vi "recurse property bag for specific properties.vi"(7 "hierarchy path":string, 10 "search key (match pattern)":string, 11 "property bag":refnum<k7>) -> (2 "matching properties":refnum<k7>[](array[refnum]), 3 "Report Text":string)   [LabVIEW 2020, in "nominal teststand model sequence support.lvlib"]
uses:
  nominal teststand model sequence support.lvlib
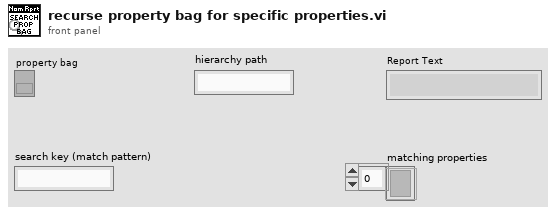
[diagram p1: front panel]
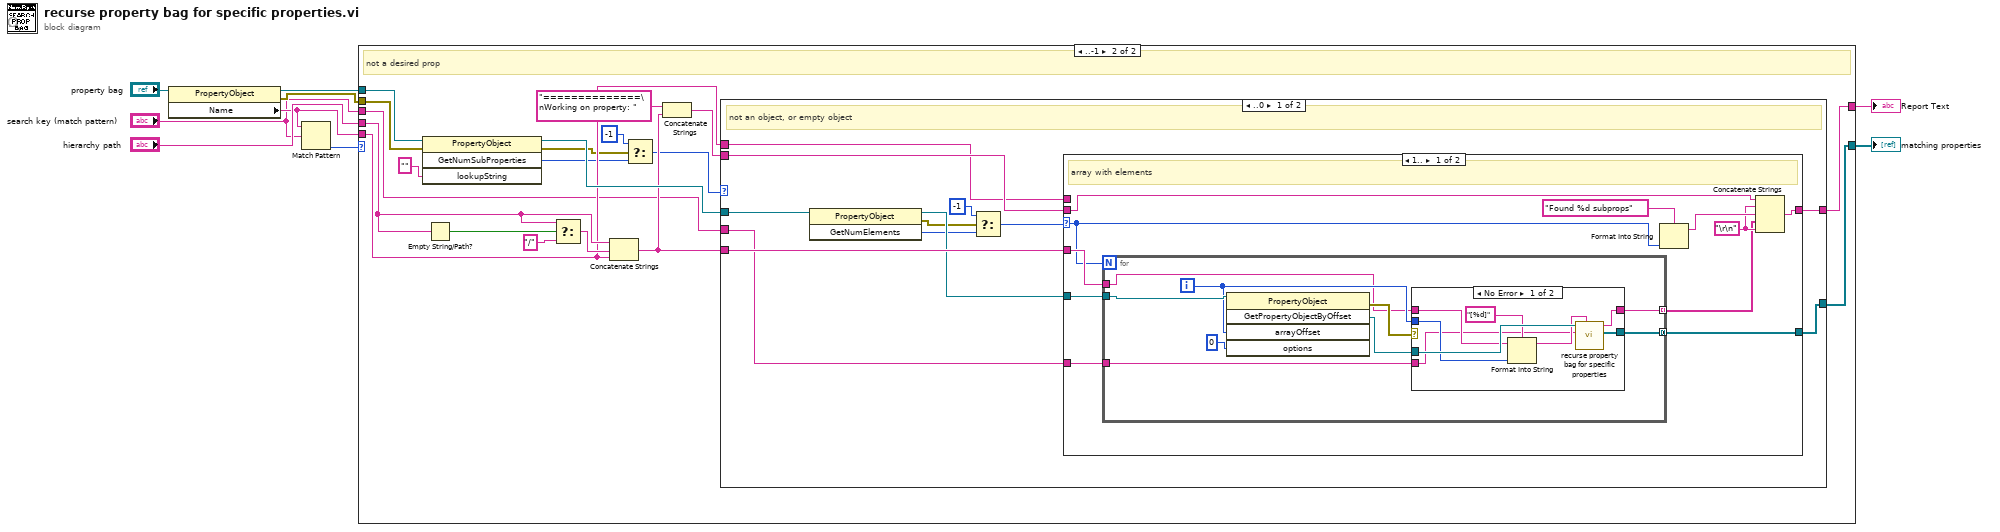
[diagram p0: block diagram]
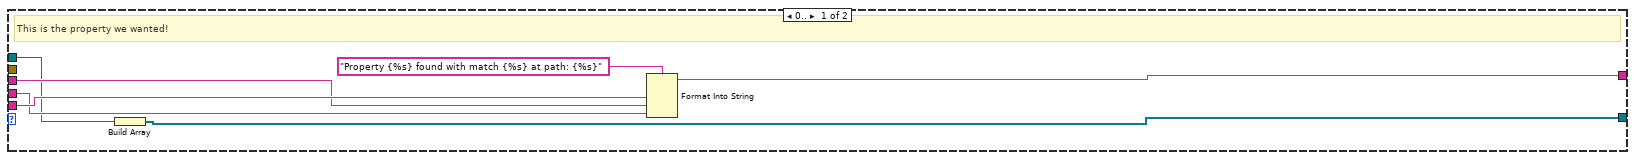
[diagram p2: hidden frame]
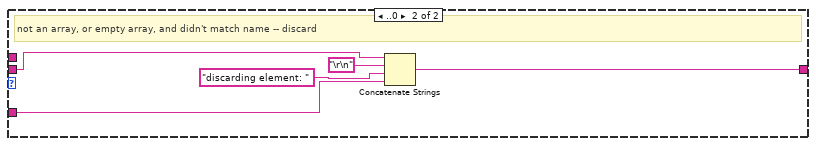
[diagram p4: hidden frame]
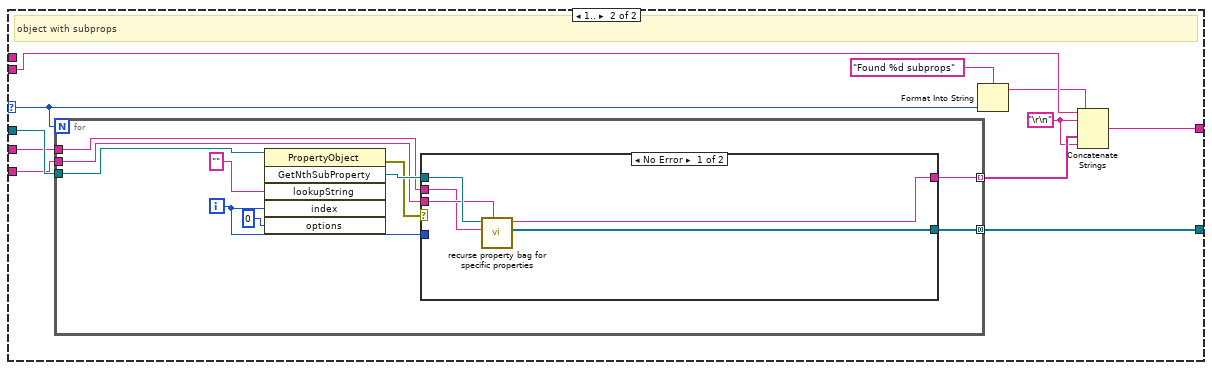
[diagram p5: hidden frame]
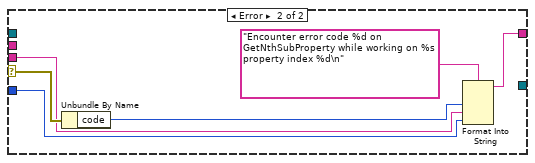
[diagram p6: hidden frame]
diagram:
  n1 = property class="PropertyObject"(reference="property bag") -> (reference out=w7:refnum<k7>, error out=w8:errorcluster, "Name"=w4:string)  [unwired: 1 in]
  n2 = Match Pattern(string=w4, regular expression="search key (match pattern)") -> (offset past match=w3:i32)  [unwired: 1 in, 3 out]
  n3 = case shown="..-1" w3 {
    tunnel: w8 -> [_ w33]
    tunnel: w7 -> [w11 w32]
    tunnel: [w12 w29] -> w6
    tunnel: "hierarchy path" -> [w14 w26]
    tunnel: w4 -> [w16 w23]
    tunnel: "search key (match pattern)" -> [w15 w18]
    tunnel: [w10 w17] -> w1
    frame 0.. {
      # "This is the property we wanted!"
      n4 = Build Array(w11) -> (w10:refnum<k7>[])
      n5 = Format Into String(format string="Property {%s} found with match {%s} at path: {%s}", w16, w15, w14) -> (resulting string=w12:string)  [unwired: 2 in, 1 out]
    }
    frame ..-1 {
      # "not a desired prop"
      n6 = invoke class="PropertyObject" method="GetNumSubProperties"(reference=w32, error in=w33, "lookupString"="") -> (reference out=w35:refnum<k7>, error out=w22:errorcluster, "GetNumSubProperties"=w21:i32)  [unwired: 1 in, 1 out]
      n7 = Empty String/Path?(string/path=w26) -> (empty?=w27:bool)
      n8 = Select(t=w26, s=w27, f="/" ("string")) -> (s? t:f=w24:string)
      n9 = Concatenate Strings(w26, w24, w23) -> (w28:string)
      n10 = Select(t=-1, s=w22, f=w21) -> (s? t:f=w19:i32)
      n11 = Concatenate Strings("==============\nWorking on property: " ("string"), w28) -> (w30:string)
      n12 = case shown="..0" w19 {
        selector: w19 -> [_ w88]
        tunnel: w35 -> [w44 w91]
        tunnel: w28 -> [w47 w83]
        tunnel: w30 -> [w45 w90]
        tunnel: [w46 w86] -> w29
        tunnel: w23 -> [w38 _]
        tunnel: w18 -> [w37 w82]
        tunnel: [w36 w81] -> w17
        frame ..0 {
          # "not an object, or empty object"
          n13 = invoke class="PropertyObject" method="GetNumElements"(reference=w44) -> (reference out=w43:refnum<k7>, error out=w42:errorcluster, "GetNumElements"=w41:i32)  [unwired: 2 in]
          n14 = Select(t=-1, s=w42, f=w41) -> (s? t:f=w39:i32)
          n15 = case shown="1.." w39 {
            selector: w39 -> [w51 _]
            tunnel: w47 -> [w57 w76]
            tunnel: [w53 w80] -> w46
            tunnel: w45 -> [w52 w79]
            tunnel: w43 -> [w58 _]
            tunnel: w38 -> [_ _]
            tunnel: w37 -> [w49 _]
            tunnel: [w48 _] -> w36
            frame 1.. {
              w54 = "\r\n"
              # "array with elements"
              n16 = for {
                N: w51 -> [_]
                tunnel: w58 -> [w67]
                tunnel: w57 -> [w62]
                tunnel: [w61] -> w50 mode=indexing
                tunnel: w49 -> [w60]
                tunnel: [w59] -> w48 mode=concatenating
                i -> [w63]
                n17 = invoke class="PropertyObject" method="GetPropertyObjectByOffset"(reference=w67, "arrayOffset"=w63, "options"=0) -> (error out=w64:errorcluster, "GetPropertyObjectByOffset"=w65:refnum<k7>)  [unwired: 2 in, 3 out]
                n18 = case shown="No Error" w64 {
                  tunnel: w65 -> [w75 _]
                  tunnel: w63 -> [w73 _]
                  tunnel: w62 -> [w72 _]
                  tunnel: [w70 _] -> w61
                  tunnel: w60 -> [w69 _]
                  tunnel: [w68 _] -> w59
                  frame No Error {
                    n19 = Format Into String(format string="[%d]", initial string=w72, w73) -> (resulting string=w74:string)  [unwired: 1 in, 1 out]
                    n20 = call "recurse property bag for specific properties.vi"("hierarchy path"=w74, "search key (match pattern)"=w69, "property bag"=w75) -> ("matching properties"=w68:refnum<k7>[], "Report Text"=w70:string)  [unwired: 7 in]
                  }
                  frame Error {
                  }
                }
              }
              n21 = Format Into String(format string="Found %d subprops", w51) -> (resulting string=w56:string)  [unwired: 2 in, 1 out]
              n22 = Concatenate Strings(w52, w54, w56, w50, w54) -> (w53:string)
            }
            frame ..0 {
              # "not an array, or empty array, and didn't match name -- discard"
              n23 = Concatenate Strings(w79, "\r\n", "discarding element: " ("string"), w76) -> (w80:string)
            }
          }
        }
        frame 1.. {
          w84 = "\r\n"
          # "object with subprops"
          n24 = for {
            N: w88 -> [_]
            tunnel: w91 -> [w101]
            tunnel: [w96] -> w85 mode=indexing
            tunnel: w83 -> [w94]
            tunnel: w82 -> [w93]
            tunnel: [w92] -> w81 mode=concatenating
            i -> [w95]
            n25 = invoke class="PropertyObject" method="GetNthSubProperty"(reference=w101, "lookupString"="", "index"=w95, "options"=0) -> (error out=w97:errorcluster, "GetNthSubProperty"=w98:refnum<k7>)  [unwired: 2 in, 4 out]
            n26 = case shown="No Error" w97 {
              selector: w97 -> [_ w110]
              tunnel: w98 -> [w106 _]
              tunnel: [w105 w111] -> w96
              tunnel: w95 -> [_ w108]
              tunnel: w94 -> [w104 w107]
              tunnel: w93 -> [w103 _]
              tunnel: [w102 _] -> w92
              frame No Error {
                n27 = call "recurse property bag for specific properties.vi"("hierarchy path"=w104, "search key (match pattern)"=w103, "property bag"=w106) -> ("matching properties"=w102:refnum<k7>[], "Report Text"=w105:string)  [unwired: 7 in]
              }
              frame Error {
                n28 = Unbundle By Name(w110) -> ("code"=w109:i32)
                n29 = Format Into String(format string="Encounter error code %d on GetNthSubProperty while working on %s property index %d\n", w109, w107, w108) -> (resulting string=w111:string)  [unwired: 2 in, 1 out]
              }
            }
          }
          n30 = Format Into String(format string="Found %d subprops", w88) -> (resulting string=w89:string)  [unwired: 2 in, 1 out]
          n31 = Concatenate Strings(w90, w84, w89, w85, w84) -> (w86:string)
        }
      }
    }
  }
  "Report Text" <- w6
  "matching properties" <- w1
